vi "Ecrire config EDWARDS.vi"(2 "error in (no error)":errorcluster caption="entrée d'erreur (pas d'erreur)", 3 "refnum":T2) -> (0 "error out":errorcluster, 1 "refnum out":T2)   [LabVIEW 2022 SP3]
uses:
  <vilib>/Utility/config.llb/Config Data RefNum.ctl
  Gestion grappe/TypeDef_Seuil Jauge Pression_CN.ctl
  Variables globales/Variable glob Edwards.vi
  <vilib>/Utility/config.llb/Write Key (String).vi
  <vilib>/Utility/config.llb/Write Key (Boolean).vi
  <vilib>/Utility/config.llb/NI_LVConfig.lvlib
panel:
  out "Seuil Jauge":T1={"Descente en Pression"={"Min Mesure Piezo"=5.0, "Min Mesure Pirani"=0.0002}, "Montée en Pression"={"Max Mesure Pirani"=10.0, "Max Mesure Penning"=0.0004}} {"Montée en Pression"."Max Mesure Penning" format="%.2e"; "Montée en Pression"."Max Mesure Pirani" format="%.2e"; "Descente en Pression"."Min Mesure Pirani" format="%.2e"; "Descente en Pression"."Min Mesure Piezo" format="%.2e"}
  out "Sélect Grappes":bool[](array[boolean])
  out "Grappes":string[][](array[string])
  out "Sélect Edwards":bool[][](array[boolean])
  out "Ports COM EDWARDS":refnum<visa-resource-name>[](array[refnum])
  out "Voies EDWARDS":u8[][](array[numeric])=[[1, 1], [1, 0]] max=6
  out "Noms jauges":string[][](array[string])
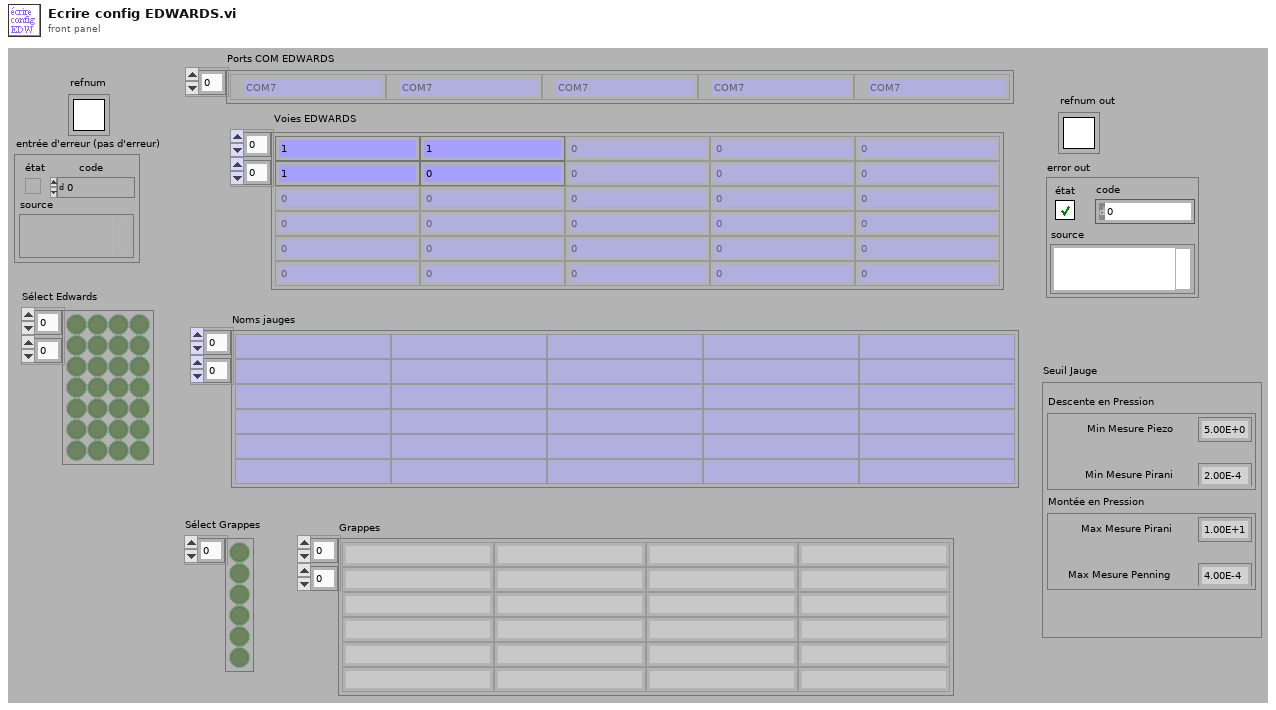
[diagram p1: front panel]
types:
  T1 = typedef "TypeDef_Seuil Jauge Pression_CN.ctl" = cluster{"Descente en Pression":cluster{"Min Mesure Piezo":dbl, "Min Mesure Pirani":dbl}, "Montée en Pression":cluster{"Max Mesure Pirani":dbl, "Max Mesure Penning":dbl}}
  T2 = typedef "NI_LVConfig.lvlib/Config Data RefNum.ctl" = refnum<k1>
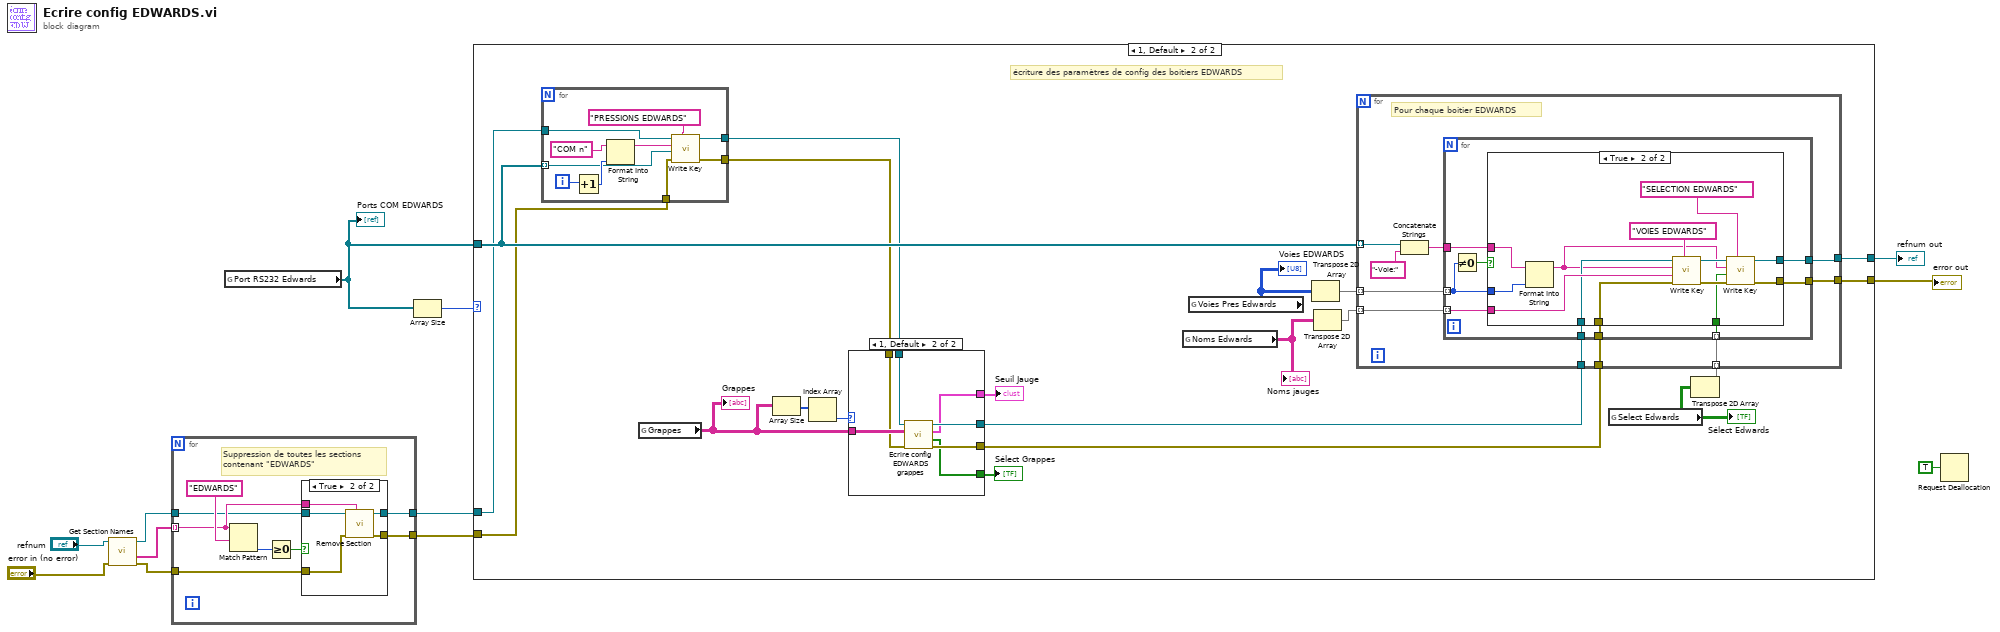
[diagram p0: block diagram]
diagram:
  n1 = call <vilib>:"Get Section Names.vi"("error in (no error)"="error in (no error)", "refnum"="refnum") -> ("error out"=w7:errorcluster, "section names"=w9:string[], "refnum out"=w8:T2)  [unwired: 7 in]
  n2 = for {
    tunnel: w9 -> [w17] mode=indexing
    tunnel: w8 -> [w16]
    tunnel: w7 -> [w15]
    tunnel: [w14] -> w4
    tunnel: [w13] -> w3
    # "Suppression de toutes les sections\ncontenant \"EDWARDS\""
    n3 = Match Pattern(string=w17, regular expression="EDWARDS" ("expression régulière")) -> (offset past match=w19:i32)  [unwired: 1 in, 3 out]
    n4 = Greater Or Equal To 0?(x=w19) -> (x >= 0?=w18:bool)
    n5 = case shown="True" w18 {
      tunnel: w17 -> [_ w27]
      tunnel: w16 -> [w22 w26]
      tunnel: w15 -> [w21 w25]
      tunnel: [w22 w24] -> w14
      tunnel: [w21 w23] -> w13
      frame False {
      }
      frame True {
        n6 = call <vilib>:"Remove Section.vi"("section"=w27, "error in (no error)"=w25, "refnum"=w26) -> ("error out"=w23:errorcluster, "refnum out"=w24:T2)  [unwired: 6 in, 1 out]
      }
    }
  }
  n7 = global read "Variable glob Edwards.vi" "Port RS232 Edwards"() -> (w2:refnum<visa-resource-name>[])
  "Ports COM EDWARDS" <- w2
  n8 = Array Size(array=w2) -> (size(s)=w10:i32)
  n9 = case shown="1, Default" w10 {
    tunnel: w3 -> [w28 w39]
    tunnel: w4 -> [w29 w40]
    tunnel: [w29 w47] -> w12
    tunnel: [w28 w46] -> w11
    tunnel: w2 -> [_ w45]
    frame 0 {
      # "Pas de boitier EDWARDS"
    }
    frame 1, Default {
      # "écriture des paramètres de config des boitiers EDWARDS"
      n10 = for {
        tunnel: w45 -> [w99] mode=indexing
        tunnel: w40 -> [w97]
        tunnel: w39 -> [w96]
        tunnel: [w95] -> w35
        tunnel: [w94] -> w38
        i -> [w102]
        n11 = Increment(x=w102) -> (x+1=w101:i32)
        n12 = Format Into String(initial string="COM n", w101) -> (resulting string=w100:string)  [unwired: 2 in, 1 out]
        n13 = call-poly <vilib>:"Write Key.vi"("section"="PRESSIONS EDWARDS", "error in (no error)"=w96, "value"=w99, "key"=w100, "refnum"=w97) -> ("error out"=w94:errorcluster, "refnum out"=w95:T2)  [unwired: 4 in, 1 out]
      }
      n14 = global read "Variable glob Edwards.vi" "Grappes"() -> (w32:string[][])
      "Grappes" <- w32
      n15 = Array Size(array=w32) -> (size(s)=w31:i32[])
      n16 = Index Array(array=w31) -> (element=w30:i32)  [unwired: 1 in]
      n17 = case shown="1, Default" w30 {
        tunnel: w32 -> [_ w58]
        tunnel: w38 -> [w50 w57]
        tunnel: [w51 w56] -> w37
        tunnel: [w50 w55] -> w36
        tunnel: w35 -> [w51 w54]
        tunnel: [_ w53] -> w34
        tunnel: [_ w52] -> w33
        frame 0 {
        }
        frame 1, Default {
          n18 = call "Ecrire config EDWARDS grappes.vi"("entrée d'erreur (pas d'erreur)"=w57, "Grappes"=w58, "Refnum en entrée"=w54) -> ("sortie d'erreur"=w55:errorcluster, "Sélect Grappes"=w52:bool[], "Seuil Jauge"=w53:T1, "Refnum en sortie"=w56:T2)  [unwired: 5 in]
        }
      }
      "Sélect Grappes" <- w33
      "Seuil Jauge" <- w34
      n19 = global read "Variable glob Edwards.vi" "Noms Edwards"() -> (w44:string[][])
      "Noms jauges" <- w44
      n20 = global read "Variable glob Edwards.vi" "Voies Pres Edwards"() -> (w43:i8[][])
      "Voies EDWARDS" <- w43
      n21 = Transpose 2D Array(2D array=w43) -> (transposed array=w48:i8[][])
      n22 = Transpose 2D Array(2D array=w44) -> (transposed array=w49:string[][])
      n23 = global read "Variable glob Edwards.vi" "Select Edwards"() -> (w42:bool[][])
      "Sélect Edwards" <- w42
      n24 = Transpose 2D Array(2D array=w42) -> (transposed array=w41:bool[][])
      n25 = for {
        tunnel: w45 -> [w65] mode=indexing
        tunnel: w48 -> [w68] mode=indexing
        tunnel: w49 -> [w67] mode=indexing
        tunnel: w37 -> [w63]
        tunnel: w36 -> [w62]
        tunnel: [w61] -> w46
        tunnel: [w60] -> w47
        tunnel: w41 -> [w59] mode=indexing
        # "Pour chaque boitier EDWARDS"
        n26 = Concatenate Strings(w65, "-Voie:") -> (w64:string)
        n27 = for {
          tunnel: w68 -> [w72] mode=indexing
          tunnel: w67 -> [w76] mode=indexing
          tunnel: w64 -> [w77]
          tunnel: w63 -> [w75]
          tunnel: w62 -> [w74]
          tunnel: [w71] -> w61
          tunnel: [w70] -> w60
          tunnel: w59 -> [w69] mode=indexing
          n28 = Not Equal To 0?(x=w72) -> (x != 0?=w73:bool)
          n29 = case shown="True" w73 {
            tunnel: w77 -> [_ w81]
            tunnel: w72 -> [_ w88]
            tunnel: w76 -> [_ w91]
            tunnel: w75 -> [w78 w90]
            tunnel: w74 -> [w79 w89]
            tunnel: [w79 w83] -> w71
            tunnel: [w78 w82] -> w70
            tunnel: w69 -> [_ w80]
            frame False {
            }
            frame True {
              n30 = Format Into String(initial string=w81, w88) -> (resulting string=w84:string)  [unwired: 2 in, 1 out]
              n31 = call-poly <vilib>:"Write Key.vi"("section"="VOIES EDWARDS", "error in (no error)"=w89, "value"=w91, "key"=w84, "refnum"=w90) -> ("error out"=w86:errorcluster, "refnum out"=w87:T2)  [unwired: 4 in, 1 out]
              n32 = call-poly <vilib>:"Write Key.vi"("section"="SELECTION EDWARDS", "error in (no error)"=w86, "value"=w80, "key"=w84, "refnum"=w87) -> ("error out"=w83:errorcluster, "refnum out"=w82:T2)  [unwired: 4 in, 1 out]
            }
          }
        }
      }
    }
  }
  "refnum out" <- w12
  "error out" <- w11
  n33 = Request Deallocation(TRUE ("flag")) -> ()
